vi "Close.vi"(8 "error in":errorcluster, 9 "Stop Event":refnum<user-event>, 10 "Sequence Context":refnum<k7>, 11 "TestExec in":refnum<class "TestExec.lvclass">) -> (0 "error out":errorcluster, 3 "TestExec out":refnum<class "TestExec.lvclass">)   [LabVIEW 2025, in "TestExec.lvclass"]
uses:
  TestExec.lvclass
  TestExec.lvclass/TestExec.ctl
  <vilib>/addons/TestStand/_TSUtility.llb/TestStand - Set Property Value (Boolean).vi
  OPC UA/Abstract.lvclass
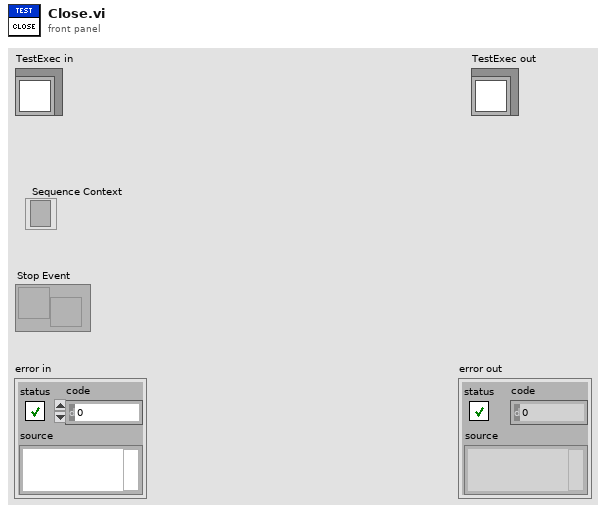
[diagram p1: front panel]
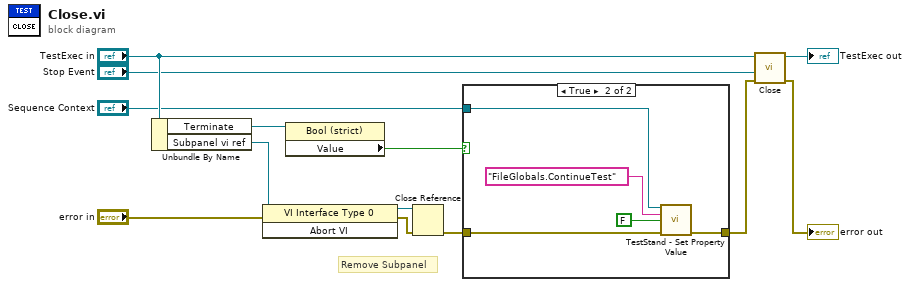
[diagram p0: block diagram]
diagram:
  # "Remove Subpanel"
  n1 = Unbundle By Name("TestExec in") -> ("Terminate"=w5:refnum<vi>, "Subpanel vi ref"=w8:refnum<vi>)
  n2 = invoke on="Invoke Node" class="VI Interface Type 0" method="Abort VI"(reference=w8, error in="error in") -> (reference out=w9:refnum<vi>, error out=w11:errorcluster)  [unwired: 1 in, 1 out]
  n3 = property class="Bool (strict)"(reference=w5) -> ("Value"=w4:bool)  [unwired: 1 in, 2 out]
  n4 = Close Reference(reference=w9, error in (no error)=w11) -> (error out=w2:errorcluster)
  n5 = case shown="True" w4 {
    tunnel: "Sequence Context" -> [_ w18]
    tunnel: w2 -> [w14 w17]
    tunnel: [w14 w16] -> w1
    frame False {
    }
    frame True {
      n6 = call-poly <vilib>:"TestStand - Set Property Value.vi"("Sequence Context In"=w18, "Lookup String"="FileGlobals.ContinueTest", "New Value"=FALSE, "error in (no error)"=w17) -> ("error out"=w16:errorcluster)  [unwired: 10 in, 1 out]
    }
  }
  n7 = call-parent "Close.vi"("error in (no error)"=w1, "Stop Event"="Stop Event", "Abstract"="TestExec in") -> ("error out"=→"error out":errorcluster, "Abstract out"=→"TestExec out":refnum<class "TestExec.lvclass">)  [unwired: 7 in]
